vi "completion complete.vi"(8 "error in":errorcluster, 10 "id":i32, 11 "message json":string) -> (0 "error out":errorcluster, 3 "response":string)   [LabVIEW 2020, in "MCP Server.lvlib"]
doc: "Handles the JSON-RPC method completion/complete (MCP utility completion, both eras). The toolkit has no source of suggestions (prompt arguments are free strings), so a known reference is answered with no values: {\"completion\":{\"values\":[],\"total\":0,\"hasMore\":false}}.\n\nparams.ref is {\"type\":\"ref/prompt\",\"name\":...} (a prompt of this server by its MCP name) or {\"type\":\"ref/resource\",\"uri\":...} (a resource of this server by its exact uri). params.argument is not checked.\n\nAnswered with JSON-RPC error -32602 (invalid params): a missing or malformed params.ref (not an object, another type, or no name or uri string in it), a prompt name this server does not have, and a uri none of its resources has. The error is built here, so error out carries only errors of the server lookup (Get Prompts.vi, Get Resources.vi) and of the response builders. The response carries id 0; Restore Request ID.vi puts the id of the request in afterwards. A modern (MCP 2026-07-28) result gets resultType and _meta in Complete Modern MCP Result.vi."
uses:
  MCP Server.lvlib
  b88a157c-7663-4469-af70-6925339ee51a.vi
  2f80e254-7019-4233-a0de-0d5826fe8f30.vi
  cb9c4109-d2d2-472b-abed-efa4ccd17b6f.vi
  <vilib>/JDP Science/JSONtext/Find Item.vi
  <vilib>/JDP Science/JSONtext/Next JSON Value.vi
  <vilib>/JDP Science/JSONtext/String Subset.vi
  <vilib>/JDP Science/JSONtext/Parsing/Advance past next JSON Value (inlined COPY).vi
  <vilib>/JDP Science/JSONtext/Parsing/Advance past whitespace.vi
  <vilib>/JDP Science/JSONtext/Parsing/Advance past String.vi
  <vilib>/JDP Science/JSONtext/Parsing/Advance past Number.vi
  <vilib>/JDP Science/JSONtext/Parsing/Advance past Line Ending.vi
  <vilib>/JDP Science/JSONtext/Parsing/Parse Full Path or Item Name.vi
  <vilib>/JDP Science/JSONtext/Parsing/Advance past Array.vi
  <vilib>/JDP Science/JSONtext/Parsing/Advance past Object.vi
  <vilib>/JDP Science/JSONtext/support/Error Cluster From Code.vi
  <vilib>/JDP Science/JSONtext/Offset/Find Item Locations by Path.vi
  <vilib>/JDP Science/JSONtext/JSON text to Variant.vi
  <vilib>/JDP Science/JSONtext/LVClass Serializer/JSONtext LVClass Serializer.lvclass
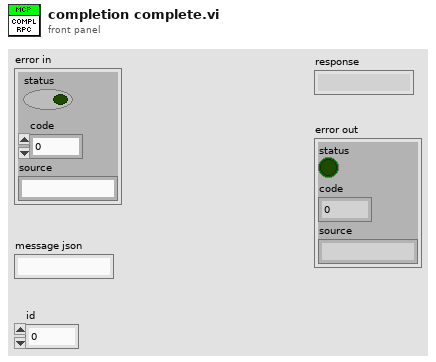
[diagram p1: front panel]
types:
  T1 = typedef "MCP Server.lvlib/Prompt Data.ctl" = cluster{"name":string, "description":string, "arguments":T2[], "return terminal name":string, "results description":string, "VI Refnum":refnum<vi>}
  T2 = typedef "MCP Server.lvlib/Prompt Argument.ctl" = cluster{"name":string, "description":string, "required":bool, "raw_name":string}
  T3 = typedef "MCP Server.lvlib/resource data.ctl" = cluster{"uri":string, "name":string, "description":string, "mimeType":string, "file path":path}
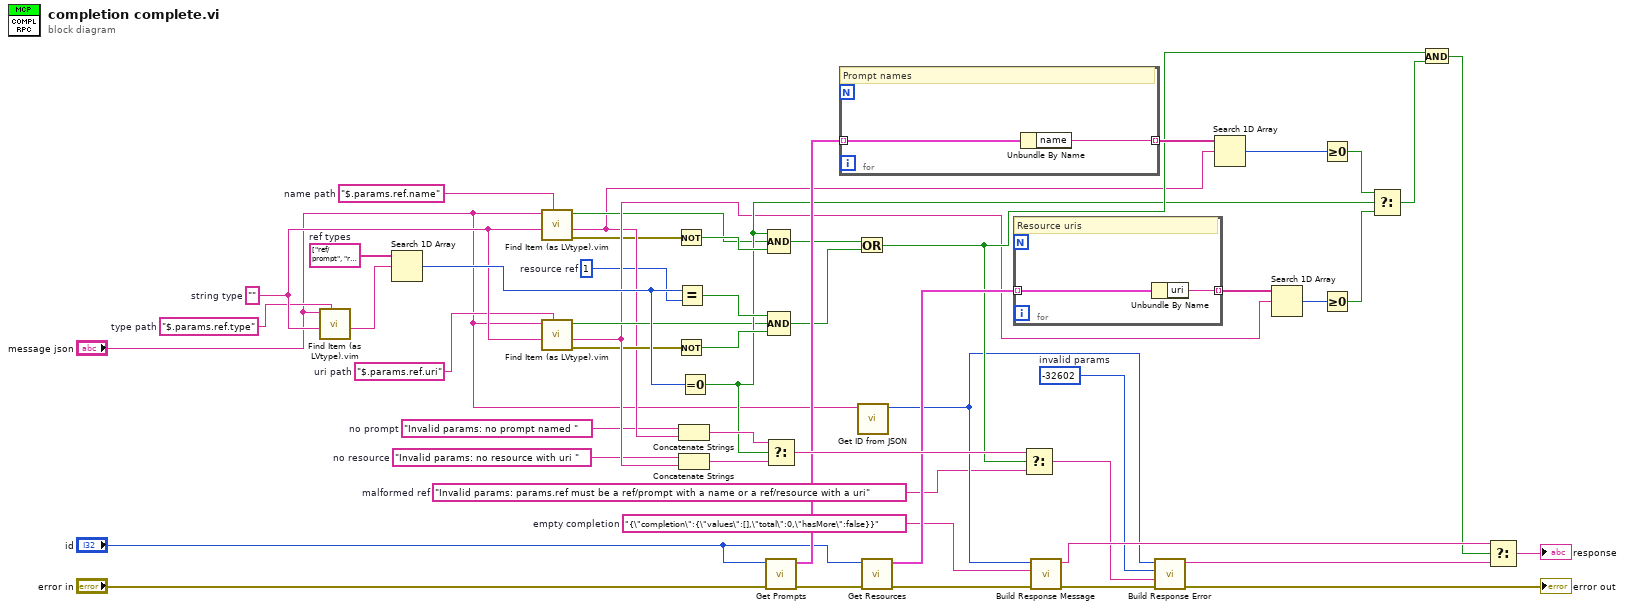
[diagram p0: block diagram]
diagram:
  w16 = "Invalid params: params.ref must be a ref/prompt with a name or a ref/resource with a uri"  # malformed ref
  w15 = "Invalid params: no resource with uri "  # no resource
  w14 = "Invalid params: no prompt named "  # no prompt
  w13 = -32602  # invalid params
  w12 = "{\"completion\":{\"values\":[],\"total\":0,\"hasMore\":false}}"  # empty completion
  w11 = 1  # resource ref
  w10 = string[] ["ref/prompt", "ref/resource"]  # ref types
  w9 = ""  # string type
  w8 = "$.params.ref.uri"  # uri path
  w7 = "$.params.ref.name"  # name path
  w6 = "$.params.ref.type"  # type path
  n1 = call "Find Item (as LVtype).vim"("$Path or Item Name"=w6, "Data Type and Default Value"=w9, "JSON"="message json") -> ("Data"=w18:string)  [unwired: 5 in, 3 out]
  n2 = Search 1D Array(1D array=w10, element=w18) -> (index of element=w25:i32)  [unwired: 1 in]
  n3 = call "Find Item (as LVtype).vim"("$Path or Item Name"=w7, "Data Type and Default Value"=w9, "JSON"="message json") -> ("error out"=w19:errorcluster, "Data"=w20:string, "Found"=w21:bool)  [unwired: 5 in, 1 out]
  n4 = call "Find Item (as LVtype).vim"("$Path or Item Name"=w8, "Data Type and Default Value"=w9, "JSON"="message json") -> ("error out"=w22:errorcluster, "Data"=w23:string, "Found"=w24:bool)  [unwired: 5 in, 1 out]
  n5 = Not(x=w19) -> (.not. x?=w28:bool)
  n6 = Not(x=w22) -> (.not. x?=w29:bool)
  n7 = Equal?(x=w25, y=w11) -> (x = y?=w27:bool)
  n8 = Concatenate Strings(w14, w20) -> (w45:string)
  n9 = Concatenate Strings(w15, w23) -> (w46:string)
  n10 = Equal To 0?(x=w25) -> (x = 0?=w26:bool)
  n11 = Select(t=w45, s=w26, f=w46) -> (s? t:f=w47:string)
  n12 = call "Get Prompts.vi"("error in (no error)"="error in", "id"="id") -> ("error out"=w33:errorcluster, "Prompts"=w34:T1[])  [unwired: 8 in]
  n13 = Compound Arithmetic op=AND(w26, w21, w28) -> (w30:bool)
  n14 = Compound Arithmetic op=AND(w27, w24, w29) -> (w31:bool)
  n15 = for {
    tunnel: w34 -> [w52] mode=indexing
    tunnel: [w53] -> w37 mode=indexing
    # "Prompt names"
    n16 = Unbundle By Name(w52) -> ("name"=w53:string)
  }
  n17 = Or(x=w30, y=w31) -> (x .or. y?=w32:bool)
  n18 = call "Get ID from JSON.vi"("message json"="message json") -> ("Data out"=w17:i32)  [unwired: 10 in]
  n19 = call "Get Resources.vi"("error in (no error)"=w33, "id"="id") -> ("error out"=w35:errorcluster, "resources"=w36:T3[])  [unwired: 8 in]
  n20 = for {
    tunnel: w36 -> [w54] mode=indexing
    tunnel: [w55] -> w38 mode=indexing
    # "Resource uris"
    n21 = Unbundle By Name(w54) -> ("uri"=w55:string)
  }
  n22 = Select(t=w47, s=w32, f=w16) -> (s? t:f=w48:string)
  n23 = call "Build Response Message.vi"("error in (no error)"=w35, "Result content"=w12, "message id in"=w17) -> ("error out"=w49:errorcluster, "MCP message out"=w50:string)  [unwired: 7 in]
  n24 = call "Build Response Error.vi"("error in (no error)"=w49, "message"=w48, "code"=w13, "message id in"=w17) -> ("error out"=→"error out":errorcluster, "MCP message out"=w51:string)  [unwired: 6 in]
  n25 = Search 1D Array(1D array=w37, element=w20) -> (index of element=w39:i32)  [unwired: 1 in]
  n26 = Search 1D Array(1D array=w38, element=w23) -> (index of element=w40:i32)  [unwired: 1 in]
  n27 = Greater Or Equal To 0?(x=w39) -> (x >= 0?=w41:bool)
  n28 = Greater Or Equal To 0?(x=w40) -> (x >= 0?=w42:bool)
  n29 = Select(t=w41, s=w26, f=w42) -> (s? t:f=w43:bool)
  n30 = And(x=w32, y=w43) -> (x .and. y?=w44:bool)
  n31 = Select(t=w50, s=w44, f=w51) -> (s? t:f=→"response":string)
